vi "Hardware In - NI 9757-1 (O2).vi"(9 "UEGOBackPressure [bar] (1.013)":sgl=1.013, 10 "Sync":bool, 11 "FPGA Ref":T1) -> (3 "O2-1":T2)   [LabVIEW 2015, in "ECS-RT.lvlib"]
uses:
  ECS-RT.lvlib
  Typedefs/Raw Inputs/NI9757.ctl
  Typedefs/FPGA Refs/Generic FPGA Ref.ctl
  <vilib>/Utility/error.llb/Error Cluster From Error Code.vi
  <vilib>/rvi/errors/niLvFpgaAdjustHostInterfaceError.vi
  <vilib>/rvi/interface/nirviReadWriteControl/nirviReadWriteControl.xnode
  <vilib>/rvi/interface/Simulation/niFpgaSimulationCallBeginRW.vi
  ECS-Shared.lvlib
  NiFpgaLv.dll
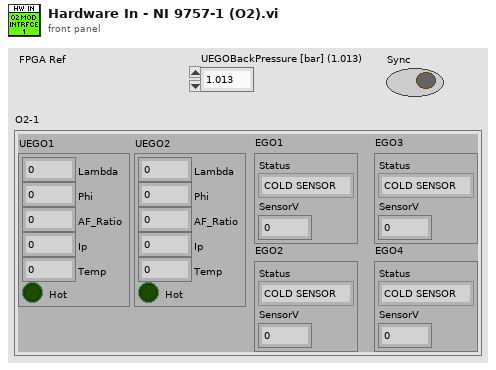
[diagram p1: front panel]
types:
  T1 = typedef "ECS-Shared.lvlib/Generic FPGA Ref.ctl" = refnum<k20>
  T2 = typedef "ECS-Shared.lvlib/NI9757.ctl" = cluster{"UEGO1":cluster{"Lambda":sgl, "Phi":sgl, "AF_Ratio":sgl, "Ip":sgl, "Temp":sgl, "Hot":bool}, "UEGO2":cluster{"Lambda":sgl, "Phi":sgl, "AF_Ratio":sgl, "Ip":sgl, "Temp":sgl, "Hot":bool}, "EGO1":cluster{"Status":enum16{"COLD SENSOR", "FOULED SENSOR", "RICH", "LEAN"}, "SensorV":sgl}, "EGO2":cluster{"Status":enum16{"COLD SENSOR", "FOULED SENSOR", "RICH", "LEAN"}, "SensorV":sgl}, "EGO3":cluster{"Status":enum16{"COLD SENSOR", "FOULED SENSOR", "RICH", "LEAN"}, "SensorV":sgl}, "EGO4":cluster{"Status":enum16{"COLD SENSOR", "FOULED SENSOR", "RICH", "LEAN"}, "SensorV":sgl}}
  T3 = cluster{"UEGO1Enable":bool, "UEGO2Enable":bool, "EGO1Enable":bool, "EGO2Enable":bool, "EGO3Enable":bool, "EGO4Enable":bool, "UEGO1Range":bool, "UEGO2Range":bool, "FilterCutoff (Hz)":dbl}
  T4 = enum32{"Diesel", "Gasoline PFI", "Stoich GDI", "Dual Fuel"}
  T5 = cluster{"UEGO1BackPressure (bar)":sgl, "UEGO2BackPressure (bar)":sgl}
  T6 = cluster{"UEGO1Diag":u8, "UEGO2Diag":u8, "UEGO1Sensor":u16, "UEGO2Sensor":u16, "UEGO1Heater":u16, "UEGO2Heater":u16, "UEGO1AmpOffset":u16, "UEGO2AmpOffset":u16, "UEGO1RIOffset":u16, "UEGO2RIOffset":u16, "UEGO1HeaterGain":u16, "UEGO2HeaterGain":u16, "Fuse":u16, "EGO1Sensor":u16, "EGO2Sensor":u16, "EGO3Sensor":u16, "EGO4Sensor":u16, "Battery":u16, "ModulePresent":bool, "UEGO1ID":u8, "UEGO2ID":u8, "LSUType":u8}
  T7 = cluster{"Stoich A/F Ratio":sgl, "IpArray (mA)":sgl[], "LambdaArray":sgl[]}
  T8 = cluster{"ModulePresent":bool, "UEGO1SensorFault":u8, "UEGO2SensorFault":u8, "UEGO1HeaterFault":u8, "UEGO2HeaterFault":u8, "UEGOFuseStatus":u8, "Battery (V)":sgl, "LSUType":u8}
  T9 = cluster{"UEGO1Lambda":sgl, "UEGO1Phi":sgl, "UEGO1AFRatio":sgl, "UEGO1Ip (mA)":sgl, "UEGO2Lambda":sgl, "UEGO2Phi":sgl, "UEGO2AFRatio":sgl, "UEGO2Ip (mA)":sgl}
  T10 = cluster{"EGO1Status":u8, "EGO2Status":u8, "EGO3Status":u8, "EGO4Status":u8, "EGO1Sensor (V)":sgl, "EGO2Sensor (V)":sgl, "EGO3Sensor (V)":sgl, "EGO4Sensor (V)":sgl}
  T11 = cluster{"UEGO1Heater (V)":sgl, "UEGO2Heater (V)":sgl}
  T12 = cluster{"UEGO1Temp (C)":sgl, "UEGO2Temp (C)":sgl, "UEGO1Hot":bool, "UEGO2Hot":bool}
  T13 = cluster{"ModuleEnable":bool, "WatchdogIn":bool, "UEGO1Hot":bool, "UEGO2Hot":bool, "Cal1Request":bool, "Cal2Request":bool, "UEGOHeaterPeriod":u16, "UEGO1HeaterPulseWidth":u16, "UEGO2HeaterPulseWidth":u16, "UEGO1Range":bool, "UEGO2Range":bool, "LSUType (F=4.9,T=4.2)":bool}
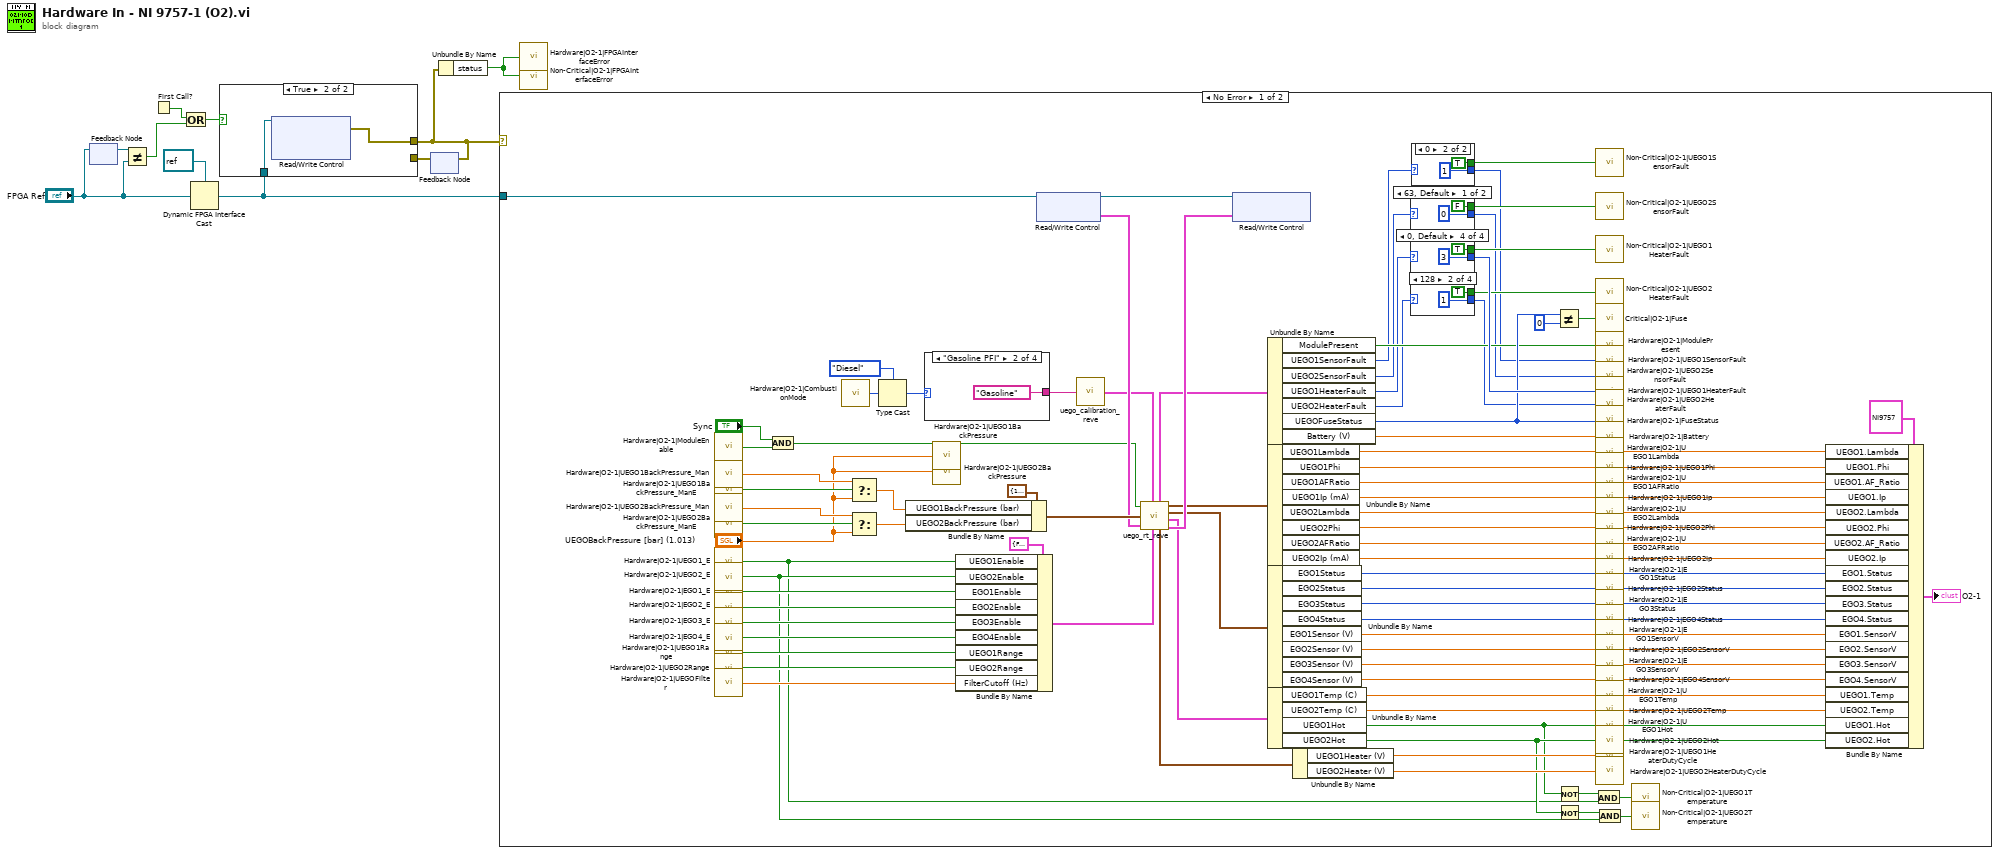
[diagram p0: block diagram]
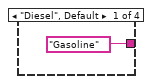
[diagram p3: hidden frame]
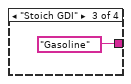
[diagram p4: hidden frame]
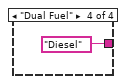
[diagram p5: hidden frame]
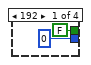
[diagram p6: hidden frame]
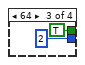
[diagram p7: hidden frame]
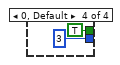
[diagram p8: hidden frame]
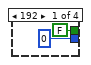
[diagram p9: hidden frame]
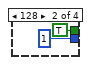
[diagram p10: hidden frame]
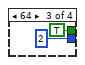
[diagram p11: hidden frame]
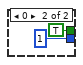
[diagram p12: hidden frame]
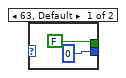
[diagram p13: hidden frame]
diagram:
  n1 = feedback #1() -> (w9:T1)  [unwired: 1 in]
  n2 = feedback-in #1("FPGA Ref") -> ()
  n3 = Not Equal?(x=w9, y="FPGA Ref") -> (x != y?=w10:bool)
  n4 = First Call?() -> (First Call?: T/F=w8:bool)
  n5 = Or(x=w8, y=w10) -> (x .or. y?=w7:bool)
  n6 = Dynamic FPGA Interface Cast(Session In=refnum<k20> refnum ("FPGA VI Reference Out"), Type="FPGA Ref") -> (Session Out=w3:refnum<k20>)
  n7 = feedback #2() -> (w6:errorcluster)  [unwired: 1 in]
  n8 = case shown="True" w7 {
    tunnel: [w11 w13] -> w2
    tunnel: w6 -> [w11 _]
    tunnel: w3 -> [_ w12]
    frame False {
    }
    frame True {
      n9 = xnode "Read/Write Control"("FPGA VI Reference In"=w12) -> ("error out"=w13:errorcluster)  [unwired: 2 in, 2 out]
    }
  }
  n10 = feedback-in #2(w2) -> ()
  n11 = Unbundle By Name(w2) -> ("status"=w1:bool)
  n12 = case shown="No Error" w2 {
    tunnel: w3 -> [w42 _]
    frame No Error {
      n13 = call "Hardware|O2-1|ModuleEnable"() -> ("Value"=w16:bool)
      n14 = call "Hardware|O2-1|UEGO1BackPressure_Man"() -> ("Value"=w84:sgl)
      n15 = call "Hardware|O2-1|UEGO1BackPressure_ManE"() -> ("Value"=w81:bool)
      n16 = call "Hardware|O2-1|UEGO2BackPressure_Man"() -> ("Value"=w83:sgl)
      n17 = call "Hardware|O2-1|UEGO2BackPressure_ManE"() -> ("Value"=w82:bool)
      n18 = call "Hardware|O2-1|UEGO1_E"() -> ("Value"=w17:bool)
      n19 = call "Hardware|O2-1|UEGO2_E"() -> ("Value"=w18:bool)
      n20 = call "Hardware|O2-1|EGO1_E"() -> ("Value"=w75:bool)
      n21 = call "Hardware|O2-1|EGO2_E"() -> ("Value"=w76:bool)
      n22 = call "Hardware|O2-1|EGO3_E"() -> ("Value"=w77:bool)
      n23 = call "Hardware|O2-1|EGO4_E"() -> ("Value"=w78:bool)
      n24 = call "Hardware|O2-1|UEGO1Range"() -> ("Value"=w21:bool)
      n25 = call "Hardware|O2-1|UEGO2Range"() -> ("Value"=w23:bool)
      n26 = call "Hardware|O2-1|UEGOFilter"() -> ("Value"=w22:sgl)
      n27 = And(x="Sync", y=w16) -> (x .and. y?=w15:bool)
      n28 = call "Hardware|O2-1|CombustionMode"() -> ("Value"=w44:u32)
      n29 = Select(t=w84, s=w81, f="UEGOBackPressure [bar] (1.013)") -> (s? t:f=w80:sgl)
      n30 = Select(t=w83, s=w82, f="UEGOBackPressure [bar] (1.013)") -> (s? t:f=w79:sgl)
      n31 = Type Cast(type=T4."Diesel" ("CombustionMode"), x=w44) -> (*(type *) &x=w43:T4)
      n32 = Bundle By Name(cluster=T5 {"UEGO1BackPressure (bar)"=1.013, "UEGO2BackPressure (bar)"=1.013} ("UEGO Back Pressure (bar)"), "UEGO1BackPressure (bar)"=w80, "UEGO2BackPressure (bar)"=w79) -> (w68:T5)
      n33 = case shown="\"Gasoline PFI\"" w43 {
        tunnel: ["Gasoline" ("Fuel Selection UEGO") "Gasoline" ("Fuel Selection UEGO") "Gasoline" ("Fuel Selection UEGO") "Diesel" ("Fuel Selection UEGO")] -> w57
        frame "Diesel", Default {
        }
        frame "Gasoline PFI" {
        }
        frame "Stoich GDI" {
        }
        frame "Dual Fuel" {
        }
      }
      n34 = call "Hardware|O2-1|UEGO1BackPressure"("Value"="UEGOBackPressure [bar] (1.013)") -> ()
      n35 = call "Hardware|O2-1|UEGO2BackPressure"("Value"="UEGOBackPressure [bar] (1.013)") -> ()
      n36 = Bundle By Name(cluster=T3 {"UEGO1Enable"=FALSE, "UEGO2Enable"=FALSE, "EGO1Enable"=FALSE, "EGO2Enable"=FALSE, "EGO3Enable"=FALSE, "EGO4Enable"=FALSE, "UEGO1Range"=FALSE, "UEGO2Range"=FALSE, "FilterCutoff (Hz)"=10.0} ("SensorControl"), "UEGO1Enable"=w17, "UEGO2Enable"=w18, "EGO1Enable"=w75, "EGO2Enable"=w76, "EGO3Enable"=w77, "EGO4Enable"=w78, "UEGO1Range"=w21, "UEGO2Range"=w23, "FilterCutoff (Hz)"=w22) -> (w24:T3)
      n37 = xnode "Read/Write Control"("FPGA VI Reference In"=w42) -> ("FPGA VI Reference Out"=w61:refnum<k20>, "O2-1.Data"=w60:T6)  [unwired: 1 in, 1 out]
      n38 = call <vilib>:"uego_calibration_reve.vi"("Fuel Selection"=w57) -> ("UEGOCalibration"=w58:T7)
      n39 = call <vilib>:"uego_rt_reve.vi"("UEGOModuleEnable"=w15, "UEGOCalibration"=w58, "UEGO Back Pressure (bar)"=w68, "UEGOData (From FPGA)"=w60, "SensorControl"=w24) -> ("UEGO Diagnostics"=w63:T8, "UEGO Sensor Results"=w62:T9, "EGO Sensor Results"=w64:T10, "UEGO Heater (V)"=w66:T11, "UEGO Temperature (C)"=w65:T12, "UEGOControl (To FPGA)"=w95:T13)
      n40 = xnode "Read/Write Control"("FPGA VI Reference In"=w61, "O2-1.Control"=w95) -> ()  [unwired: 1 in, 2 out]
      n41 = Unbundle By Name(w63) -> ("ModulePresent"=w88:bool, "UEGO1SensorFault"=w54:u8, "UEGO2SensorFault"=w70:u8, "UEGO1HeaterFault"=w72:u8, "UEGO2HeaterFault"=w74:u8, "UEGOFuseStatus"=w91:u8, "Battery (V)"=w69:sgl)
      n42 = Unbundle By Name(w62) -> ("UEGO1Lambda"=w20:sgl, "UEGO1Phi"=w53:sgl, "UEGO1AFRatio"=w52:sgl, "UEGO1Ip (mA)"=w51:sgl, "UEGO2Lambda"=w19:sgl, "UEGO2Phi"=w49:sgl, "UEGO2AFRatio"=w48:sgl, "UEGO2Ip (mA)"=w47:sgl)
      n43 = Unbundle By Name(w64) -> ("EGO1Status"=w33:u8, "EGO2Status"=w32:u8, "EGO3Status"=w31:u8, "EGO4Status"=w30:u8, "EGO1Sensor (V)"=w29:sgl, "EGO2Sensor (V)"=w28:sgl, "EGO3Sensor (V)"=w27:sgl, "EGO4Sensor (V)"=w26:sgl)
      n44 = Unbundle By Name(w65) -> ("UEGO1Temp (C)"=w34:sgl, "UEGO2Temp (C)"=w35:sgl, "UEGO1Hot"=w36:bool, "UEGO2Hot"=w37:bool)
      n45 = Unbundle By Name(w66) -> ("UEGO1Heater (V)"=w93:sgl, "UEGO2Heater (V)"=w94:sgl)
      n46 = case shown="63, Default" w70 {
        tunnel: [0 1] -> w71
        tunnel: [FALSE TRUE] -> w87
        frame 63, Default {
        }
        frame 0 {
        }
      }
      n47 = case shown="0, Default" w72 {
        tunnel: [0 1 2 3] -> w92
        tunnel: [FALSE TRUE TRUE TRUE] -> w86
        frame 192 {
        }
        frame 128 {
        }
        frame 64 {
        }
        frame 0, Default {
        }
      }
      n48 = case shown="128" w74 {
        tunnel: [0 1 2 3] -> w73
        tunnel: [FALSE TRUE TRUE TRUE] -> w85
        frame 192 {
        }
        frame 128 {
        }
        frame 64 {
        }
        frame 0, Default {
        }
      }
      n49 = case shown="0" w54 {
        tunnel: [FALSE TRUE] -> w56
        tunnel: [0 1] -> w55
        frame 63, Default {
        }
        frame 0 {
        }
      }
      n50 = Not Equal?(x=w91, y=0) -> (x != y?=w90:bool)
      n51 = Not(x=w36) -> (.not. x?=w39:bool)
      n52 = Not(x=w37) -> (.not. x?=w38:bool)
      n53 = And(x=w39, y=w17) -> (x .and. y?=w40:bool)
      n54 = call "Non-Critical|O2-1|UEGO1SensorFault"("Fault"=w56) -> ()  [unwired: 2 in]
      n55 = call "Non-Critical|O2-1|UEGO2SensorFault"("Fault"=w87) -> ()  [unwired: 2 in]
      n56 = call "Non-Critical|O2-1|UEGO1HeaterFault"("Fault"=w86) -> ()  [unwired: 2 in]
      n57 = call "Non-Critical|O2-1|UEGO2HeaterFault"("Fault"=w85) -> ()  [unwired: 2 in]
      n58 = call "Critical|O2-1|Fuse"("Fault"=w90) -> ()  [unwired: 2 in]
      n59 = call "Hardware|O2-1|ModulePresent"("Value"=w88) -> ()
      n60 = call "Hardware|O2-1|UEGO1SensorFault"("Value"=w55) -> ()
      n61 = call "Hardware|O2-1|UEGO2SensorFault"("Value"=w71) -> ()
      n62 = call "Hardware|O2-1|UEGO1HeaterFault"("Value"=w92) -> ()
      n63 = call "Hardware|O2-1|UEGO2HeaterFault"("Value"=w73) -> ()
      n64 = call "Hardware|O2-1|FuseStatus"("Value"=w91) -> ()
      n65 = call "Hardware|O2-1|Battery"("Value"=w69) -> ()
      n66 = call "Hardware|O2-1|UEGO1Lambda"("Value"=w20) -> ()
      n67 = call "Hardware|O2-1|UEGO1Phi"("Value"=w53) -> ()
      n68 = call "Hardware|O2-1|UEGO1AFRatio"("Value"=w52) -> ()
      n69 = call "Hardware|O2-1|UEGO1Ip"("Value"=w51) -> ()
      n70 = call "Hardware|O2-1|UEGO2Lambda"("Value"=w19) -> ()
      n71 = call "Hardware|O2-1|UEGO2Phi"("Value"=w49) -> ()
      n72 = call "Hardware|O2-1|UEGO2AFRatio"("Value"=w48) -> ()
      n73 = call "Hardware|O2-1|UEGO2Ip"("Value"=w47) -> ()
      n74 = call "Hardware|O2-1|EGO1Status"("Value"=w33) -> ()
      n75 = call "Hardware|O2-1|EGO2Status"("Value"=w32) -> ()
      n76 = call "Hardware|O2-1|EGO3Status"("Value"=w31) -> ()
      n77 = call "Hardware|O2-1|EGO4Status"("Value"=w30) -> ()
      n78 = call "Hardware|O2-1|EGO1SensorV"("Value"=w29) -> ()
      n79 = call "Hardware|O2-1|EGO2SensorV"("Value"=w28) -> ()
      n80 = call "Hardware|O2-1|EGO3SensorV"("Value"=w27) -> ()
      n81 = call "Hardware|O2-1|EGO4SensorV"("Value"=w26) -> ()
      n82 = call "Hardware|O2-1|UEGO1Temp"("Value"=w34) -> ()
      n83 = call "Hardware|O2-1|UEGO2Temp"("Value"=w35) -> ()
      n84 = call "Hardware|O2-1|UEGO1Hot"("Value"=w36) -> ()
      n85 = call "Hardware|O2-1|UEGO2Hot"("Value"=w37) -> ()
      n86 = call "Hardware|O2-1|UEGO1HeaterDutyCycle"("Value"=w93) -> ()
      n87 = call "Hardware|O2-1|UEGO2HeaterDutyCycle"("Value"=w94) -> ()
      n88 = And(x=w38, y=w18) -> (x .and. y?=w41:bool)
      n89 = call "Non-Critical|O2-1|UEGO1Temperature"("Fault"=w40) -> ()  [unwired: 2 in]
      n90 = call "Non-Critical|O2-1|UEGO2Temperature"("Fault"=w41) -> ()  [unwired: 2 in]
      n91 = Bundle By Name(cluster=T2 {"UEGO1"={"Lambda"=0.0, "Phi"=0.0, "AF_Ratio"=0.0, "Ip"=0.0, "Temp"=0.0, "Hot"=FALSE}, "UEGO2"={"Lambda"=0.0, "Phi"=0.0, "AF_Ratio"=0.0, "Ip"=0.0, "Temp"=0.0, "Hot"=FALSE}, "EGO1"={"Status"=enum."COLD SENSOR", "SensorV"=0.0}, "EGO2"={"Status"=enum."COLD SENSOR", "SensorV"=0.0}, "EGO3"={"Status"=enum."COLD SENSOR", "SensorV"=0.0}, "EGO4"={"Status"=enum."COLD SENSOR", "SensorV"=0.0}} ("O2"), "UEGO1.Lambda"=w20, "UEGO1.Phi"=w53, "UEGO1.AF_Ratio"=w52, "UEGO1.Ip"=w51, "UEGO2.Lambda"=w19, "UEGO2.Phi"=w49, "UEGO2.AF_Ratio"=w48, "UEGO2.Ip"=w47, "EGO1.Status"=w33, "EGO2.Status"=w32, "EGO3.Status"=w31, "EGO4.Status"=w30, "EGO1.SensorV"=w29, "EGO2.SensorV"=w28, "EGO3.SensorV"=w27, "EGO4.SensorV"=w26, "UEGO1.Temp"=w34, "UEGO2.Temp"=w35, "UEGO1.Hot"=w36, "UEGO2.Hot"=w37) -> (→"O2-1":T2)
    }
    frame Error {
    }
  }
  n92 = call "Hardware|O2-1|FPGAInterfaceError"("Value"=w1) -> ()
  n93 = call "Non-Critical|O2-1|FPGAInterfaceError"("Fault"=w1) -> ()  [unwired: 2 in]
